vi "Initialization VI.vi"(8 "error in (no error)":errorcluster, 10 "Custom XML":string, 11 "Device Item Ref in":T1 format="%.0x") -> (0 "error out":errorcluster, 3 "Device Item Ref out":T1 format="%.0x")   [LabVIEW 2025, in "Protection and Counter Addon System Explorer.lvlib"]
uses:
  Protection and Counter Addon System Explorer.lvlib
  <vilib>/NI VeriStand/Custom Device API/Custom Device API.lvlib
  Addon Shared/SubVIs/GUID Lookup.vi
  Addon Shared/Protection and Counter Addon Shared.lvlib
  <vilib>/NI VeriStand/Custom Device API/Custom Device Channel Type.ctl
  <vilib>/NI VeriStand/Custom Device API/Custom Device Channel.ctl
  <vilib>/NI/NI VeriStand Custom Device Import and Export Tool/ImportExport.lvlib
  <vilib>/NI VeriStand/Custom Device API/Custom Device Item Ref.ctl
  <vilib>/NI VeriStand/Custom Device Tools/Custom Device Utility Library/Custom Device Utility Library.lvlib
  <vilib>/NI VeriStand/Custom Device Tools/Custom Device Utility Library/Search Direction.ctl
  <vilib>/NI VeriStand/Custom Device Tools/Custom Device Utility Library/NI VeriStand - Search for Item by GUID.vi
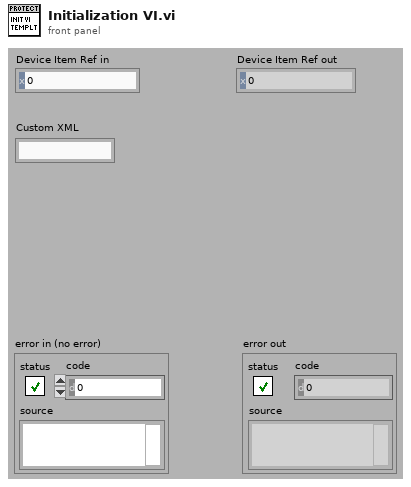
[diagram p1: front panel]
types:
  T1 = typedef "Custom Device API.lvlib/Custom Device Item Ref.ctl" = u64
  T2 = typedef "Custom Device Utility Library.lvlib/Search Direction.ctl" = enum16{"Down", "Up"}
  T3 = typedef "Custom Device API.lvlib/Custom Device Channel.ctl" = cluster{"Type":T4, "Units":string, "Default Value":dbl, "Faultable":bool, "Scalable":bool}
  T4 = typedef "Custom Device API.lvlib/Custom Device Channel Type.ctl" = enum16{"Input", "Output"}
  T5 = typedef "Protection and Counter Addon Shared.lvlib/XNET Settings.ctl" = cluster{"Database":refnum<k21>, "Cluster":refnum<k21>, "Port":string, "Baud rate [Bd]":u64, "Termination":u32, "CAN I/O Mode":u32, "FD Baud rate [Bd]":u64, "Priority":i32, "Use Legacy":bool, "FD ISO Mode":u32, "Default Max Counter Value":dbl, "Default Protect Type":T6, "Include All Channels":bool}
  T6 = typedef "Protection and Counter Support Shared.lvlib/Protection Type.ctl" = enum16{"Arb ID + Bytes Checksum with Inversion", "Arb ID + Bytes CRC with Inversion", "Reversed Raw Signal Checksum with Inversion", "Concatenated Two's Compliment"}
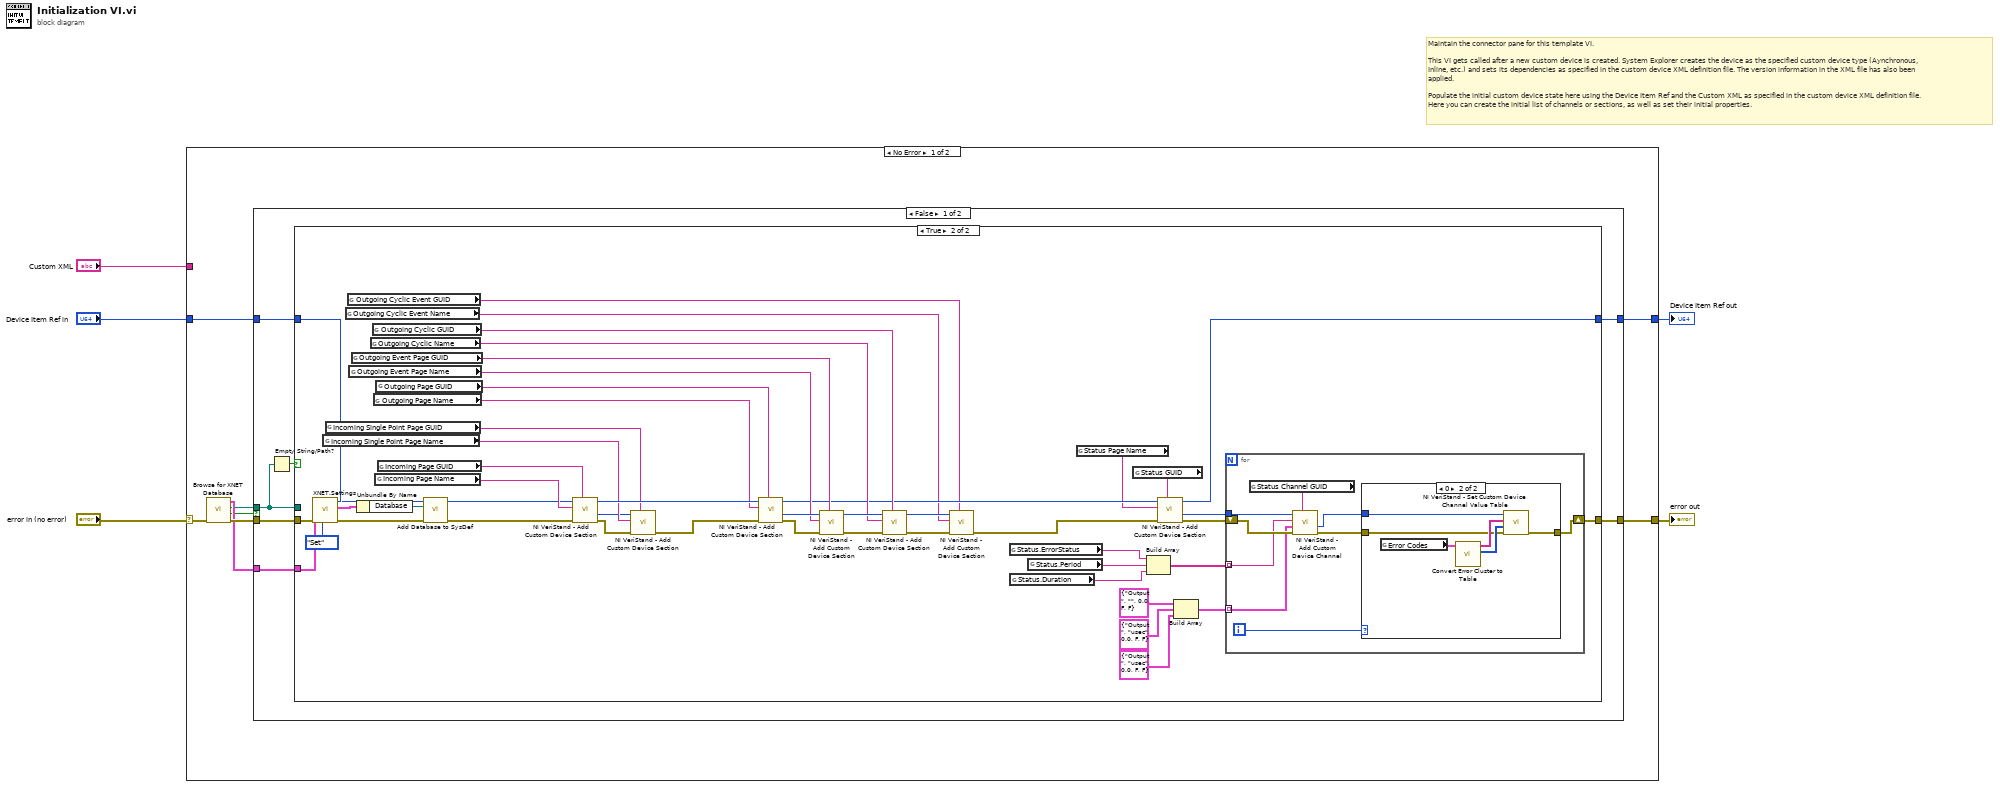
[diagram p0: block diagram]
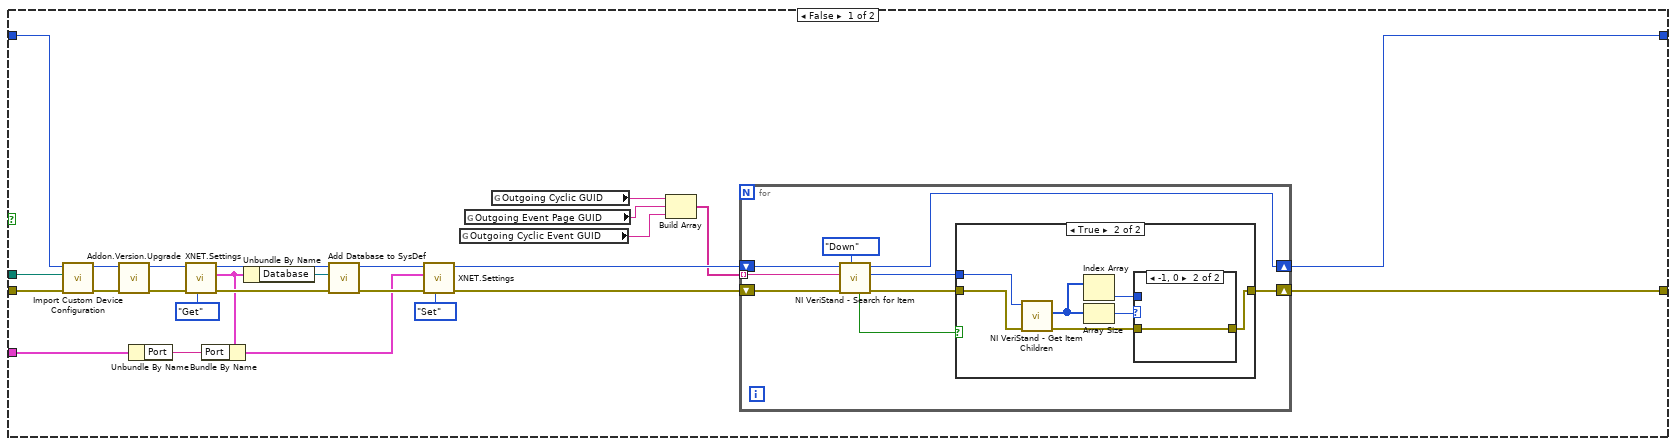
[diagram p2: hidden frame]
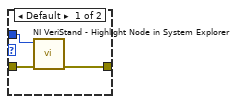
[diagram p4: hidden frame]
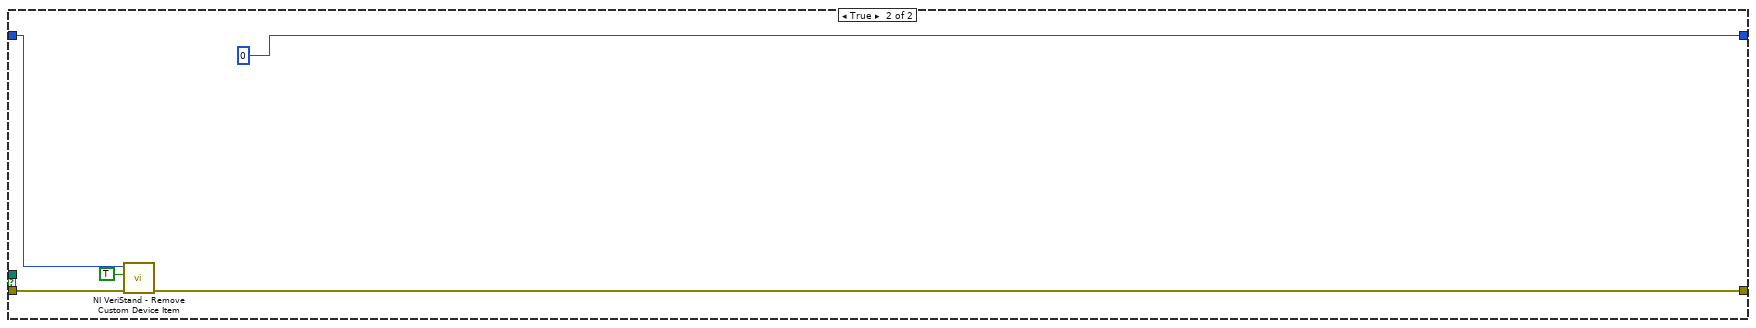
[diagram p6: hidden frame]
diagram:
  # "Maintain the connector pane for this template VI.\n\nThis VI gets called after a new custom device is created. System Explorer creates the device as the specified custom device type (Aynchronous, Inline, etc.) and sets its dependencies as specified in the custom device XML definition file. The version information in the XML file has also been applied.\n\nPopulate the initial custom device state here using the Device Item Ref and the Custom XML as specified in the custom device XML definition file. Here you can create the initial list of channels or sections, as well as set their initial properties."
  n1 = case shown="No Error" "error in (no error)" {
    selector: "error in (no error)" -> [w11 w138]
    tunnel: [w13 w138] -> w5
    tunnel: [w12 w137] -> w3
    tunnel: "Device Item Ref in" -> [w9 w137]
    tunnel: "Custom XML" -> [_ _]
    frame No Error {
      n2 = call "Browse for XNET Database.vi"("error in (no error)"=w11) -> ("error out"=w10:errorcluster, "Cancel Out"=w7:bool, "Import Path out"=w6:path, "XNET Settings"=w8:T5)  [unwired: 7 in]
      n3 = case shown="False" w7 {
        tunnel: [w16 w135] -> w13
        tunnel: [w17 T1 0 ("Parent Ref out")] -> w12
        tunnel: w10 -> [w20 w133]
        tunnel: w9 -> [w19 w132]
        tunnel: w8 -> [w18 _]
        tunnel: w6 -> [w14 _]
        frame False {
          n4 = Empty String/Path?(string/path=w14) -> (empty?=w15:bool)
          n5 = case shown="True" w15 {
            tunnel: w20 -> [w40 w108]
            tunnel: w19 -> [w46 w106]
            tunnel: w18 -> [w39 w104]
            tunnel: [w25 w86] -> w17
            tunnel: [w26 w85] -> w16
            tunnel: w14 -> [w45 _]
            frame False {
              n6 = call <vilib>:"Import Custom Device Configuration.vi"("error in (no error)"=w40, "Path"=w45, "NodeID"=w46) -> ("error out"=w44:errorcluster, "NodeID out"=w43:u64)  [unwired: 6 in, 1 out]
              n7 = call "Addon.Version.Upgrade.vi"("error in (no error)"=w44, "Device Item Ref in in"=w43) -> ("error out"=w42:errorcluster, "Device Item Ref out"=w41:T1)  [unwired: 8 in]
              n8 = Unbundle By Name(w39) -> ("Port"=w27:string)
              n9 = call "XNET.Settings.vi"("Action"=enum8{"Get", "Set"}."Get", "error in (no error)"=w42, "Parent Ref in"=w41) -> ("error out"=w37:errorcluster, "XNET Settings"=w32:T5, "Item Ref out"=w36:T1)  [unwired: 6 in]
              n10 = Bundle By Name(cluster=w32, "Port"=w27) -> (w31:T5)
              n11 = Unbundle By Name(w32) -> ("Database"=w35:refnum<k21>)
              n12 = call "Add Database to SysDef.vi"("error in"=w37, "DB Alias"=w35, "Item Ref in"=w36) -> ("error out"=w33:errorcluster, "Item Ref out"=w29:T1)  [unwired: 7 in]
              n13 = call "XNET.Settings.vi"("Action"=enum8{"Get", "Set"}."Set", "error in (no error)"=w33, "XNET Settings"=w31, "Parent Ref in"=w29) -> ("error out"=w30:errorcluster, "Item Ref out"=w28:T1)  [unwired: 5 in, 1 out]
              n14 = global read "GUID Lookup.vi" "Outgoing Cyclic Event GUID"() -> (w22:string)
              n15 = global read "GUID Lookup.vi" "Outgoing Event Page GUID"() -> (w23:string)
              n16 = global read "GUID Lookup.vi" "Outgoing Cyclic GUID"() -> (w24:string)
              n17 = Build Array(w24, w23, w22) -> (w21:string[])
              n18 = for {
                tunnel: w21 -> [w53] mode=indexing
                shift-right: [w49] -> w26
                shift-left: w30 -> [w52]
                shift-right: [w47] -> w25
                shift-left: w28 -> [w54]
                n19 = call-poly <vilib>:"NI VeriStand - Search for Item.vi"("Direction (Down)"=Search_Direction."Down", "error in"=w52, "Item GUID"=w53, "Section Ref in"=w54) -> ("error out"=w50:errorcluster, "Item Ref"=w51:T1, "Section Ref out"=w47:T1, "Found"=w48:bool)  [unwired: 4 in]
                n20 = case shown="True" w48 {
                  tunnel: w51 -> [_ w63]
                  tunnel: w50 -> [w56 w62]
                  tunnel: [w56 w57] -> w49
                  frame False {
                  }
                  frame True {
                    n21 = call <vilib>:"NI VeriStand - Get Item Children.vi"("error in (no error)"=w62, "Item Ref in"=w63) -> ("error out"=w58:errorcluster, "Child Refs"=w60:T1[])  [unwired: 6 in, 2 out]
                    n22 = Index Array(array=w60) -> (element=w59:T1)  [unwired: 1 in]
                    n23 = Array Size(array=w60) -> (size(s)=w61:i32)
                    n24 = case shown="-1, 0" w61 {
                      tunnel: w59 -> [w66 _]
                      tunnel: w58 -> [w65 w67]
                      tunnel: [w64 w67] -> w57
                      frame Default {
                        n25 = call <vilib>:"NI VeriStand - Highlight Node in System Explorer.vi"("error in (no error)"=w65, "Item Ref in"=w66) -> ("error out"=w64:errorcluster)  [unwired: 8 in, 1 out]
                      }
                      frame -1, 0 {
                      }
                    }
                  }
                }
              }
            }
            frame True {
              n26 = call "XNET.Settings.vi"("Action"=enum8{"Get", "Set"}."Set", "error in (no error)"=w108, "XNET Settings"=w104, "Parent Ref in"=w106) -> ("error out"=w107:errorcluster, "XNET Settings"=w103:T5, "Item Ref out"=w105:T1)  [unwired: 5 in]
              n27 = global read "GUID Lookup.vi" "Incoming Single Point Page Name"() -> (w90:string)
              n28 = global read "GUID Lookup.vi" "Incoming Single Point Page GUID"() -> (w91:string)
              n29 = global read "GUID Lookup.vi" "Outgoing Cyclic Event Name"() -> (w74:string)
              n30 = global read "GUID Lookup.vi" "Outgoing Cyclic Event GUID"() -> (w75:string)
              n31 = global read "GUID Lookup.vi" "Outgoing Event Page Name"() -> (w95:string)
              n32 = global read "GUID Lookup.vi" "Outgoing Event Page GUID"() -> (w96:string)
              n33 = Unbundle By Name(w103) -> ("Database"=w102:refnum<k21>)
              n34 = global read "GUID Lookup.vi" "Outgoing Cyclic Name"() -> (w93:string)
              n35 = global read "GUID Lookup.vi" "Outgoing Cyclic GUID"() -> (w94:string)
              n36 = global read "GUID Lookup.vi" "Outgoing Page Name"() -> (w112:string)
              n37 = global read "GUID Lookup.vi" "Incoming Page Name"() -> (w111:string)
              n38 = global read "GUID Lookup.vi" "Outgoing Page GUID"() -> (w113:string)
              n39 = global read "GUID Lookup.vi" "Incoming Page GUID"() -> (w115:string)
              n40 = call "Add Database to SysDef.vi"("error in"=w107, "DB Alias"=w102, "Item Ref in"=w105) -> ("error out"=w110:errorcluster, "Item Ref out"=w109:T1)  [unwired: 7 in]
              n41 = call <vilib>:"NI VeriStand - Add Custom Device Section.vi"("GUID (Default Section)"=w115, "error in (no error)"=w110, "Section Name"=w111, "Parent Ref in"=w109) -> ("error out"=w68:errorcluster, "Section Ptr"=w69:T1, "Parent Ref out"=w114:T1)  [unwired: 4 in, 1 out]
              n42 = call <vilib>:"NI VeriStand - Add Custom Device Section.vi"("GUID (Default Section)"=w91, "error in (no error)"=w68, "Section Name"=w90, "Parent Ref in"=w69) -> ("error out"=w92:errorcluster)  [unwired: 4 in, 3 out]
              n43 = call <vilib>:"NI VeriStand - Add Custom Device Section.vi"("GUID (Default Section)"=w113, "error in (no error)"=w92, "Section Name"=w112, "Parent Ref in"=w114) -> ("error out"=w98:errorcluster, "Section Ptr"=w100:T1, "Parent Ref out"=w87:T1)  [unwired: 4 in, 1 out]
              n44 = call <vilib>:"NI VeriStand - Add Custom Device Section.vi"("GUID (Default Section)"=w96, "error in (no error)"=w98, "Section Name"=w95, "Parent Ref in"=w100) -> ("error out"=w99:errorcluster, "Parent Ref out"=w97:T1)  [unwired: 4 in, 2 out]
              n45 = call <vilib>:"NI VeriStand - Add Custom Device Section.vi"("GUID (Default Section)"=w94, "error in (no error)"=w99, "Section Name"=w93, "Parent Ref in"=w97) -> ("error out"=w77:errorcluster, "Parent Ref out"=w78:T1)  [unwired: 4 in, 2 out]
              n46 = call <vilib>:"NI VeriStand - Add Custom Device Section.vi"("GUID (Default Section)"=w75, "error in (no error)"=w77, "Section Name"=w74, "Parent Ref in"=w78) -> ("error out"=w76:errorcluster)  [unwired: 4 in, 3 out]
              n47 = global read "GUID Lookup.vi" "Status.ErrorStatus"() -> (w84:string)
              n48 = global read "GUID Lookup.vi" "Status.Duration"() -> (w82:string)
              n49 = global read "GUID Lookup.vi" "Status.Period"() -> (w83:string)
              n50 = global read "GUID Lookup.vi" "Status Page Name"() -> (w79:string)
              n51 = global read "GUID Lookup.vi" "Status GUID"() -> (w80:string)
              n52 = Build Array(w84, w83, w82) -> (w81:string[])
              n53 = call <vilib>:"NI VeriStand - Add Custom Device Section.vi"("GUID (Default Section)"=w80, "error in (no error)"=w76, "Section Name"=w79, "Parent Ref in"=w87) -> ("error out"=w88:errorcluster, "Section Ptr"=w89:T1, "Parent Ref out"=w86:T1)  [unwired: 4 in, 1 out]
              n54 = Build Array(T3 {"Type"=enum."Output", "Units"="", "Default Value"=0.0, "Faultable"=FALSE, "Scalable"=FALSE} ("Channel"), T3 {"Type"=enum."Output", "Units"="usec", "Default Value"=0.0, "Faultable"=FALSE, "Scalable"=FALSE} ("Channel"), T3 {"Type"=enum."Output", "Units"="usec", "Default Value"=0.0, "Faultable"=FALSE, "Scalable"=FALSE} ("Channel")) -> (w70:T3[])
              n55 = for {
                tunnel: w89 -> [w124]
                shift-right: [w117] -> w85
                shift-left: w88 -> [w123]
                tunnel: w81 -> [w121] mode=indexing
                tunnel: w70 -> [w120] mode=indexing
                i -> [w119]
                n56 = global read "GUID Lookup.vi" "Status Channel GUID"() -> (w122:string)
                n57 = call <vilib>:"NI VeriStand - Add Custom Device Channel.vi"("GUID (Default Channel)"=w122, "error in (no error)"=w123, "Channel"=w120, "Channel Name"=w121, "Parent Ref in"=w124) -> ("error out"=w118:errorcluster, "Channel Ref"=w116:T1)  [unwired: 3 in, 2 out]
                n58 = case shown="0" w119 {
                  tunnel: w116 -> [_ w130]
                  tunnel: w118 -> [w125 w127]
                  tunnel: [w125 w126] -> w117
                  frame Default {
                  }
                  frame 0 {
                    n59 = global read "GUID Lookup.vi" "Error Codes"() -> (w131:cluster{"number":i32, "trimmed string":string}[])
                    n60 = call "Convert Error Cluster to Table.vi"("Error Codes"=w131) -> ("Code"=w128:i32[], "String"=w129:string[])  [unwired: 9 in]
                    n61 = call <vilib>:"NI VeriStand - Set Custom Device Channel Value Table.vi"("error in (no error)"=w127, "Values"=w128, "Names"=w129, "Channel Ref in"=w130) -> ("error out"=w126:errorcluster)  [unwired: 6 in, 1 out]
                  }
                }
              }
            }
          }
        }
        frame True {
          n62 = call <vilib>:"NI VeriStand - Remove Custom Device Item.vi"("error in (no error)"=w133, "Force Delete (F)"=TRUE, "Item Ref in"=w132) -> ("error out"=w135:errorcluster)  [unwired: 7 in, 1 out]
        }
      }
    }
    frame Error {
    }
  }
  "error out" <- w5
  "Device Item Ref out" <- w3
